vi "Create Oneof Protobuf To Field Name.vi"(8 "error in (no error)":errorcluster, 10 "message element metadata":T1={"Field Name"="nested_message_2", "Embedded Message Name"="echo_array_NestedMessage2", "Protobuf Index"=3, "MessageElementType"=enum."MessageValue", "Repeated"=FALSE, "Is in Oneof"=TRUE, "Oneof Container Name"="echo_array_NestedMessage_union"}, 11 "class in":refnum<vi>) -> (0 "error out":errorcluster, 3 "class out":refnum<vi>)   [LabVIEW 2019, in "gRPC Template Creation Utility.lvlib"]
uses:
  gRPC Template Creation Utility.lvlib
  TypeDefs/Message Element Metadata (Scripting).ctl
  TypeDefs/Message Element Type.ctl
  <vilib>/Utility/traverseref.llb/TRef TravTarget.ctl
  <vilib>/Utility/traverseref.llb/VI Scripting - Traverse.lvlib
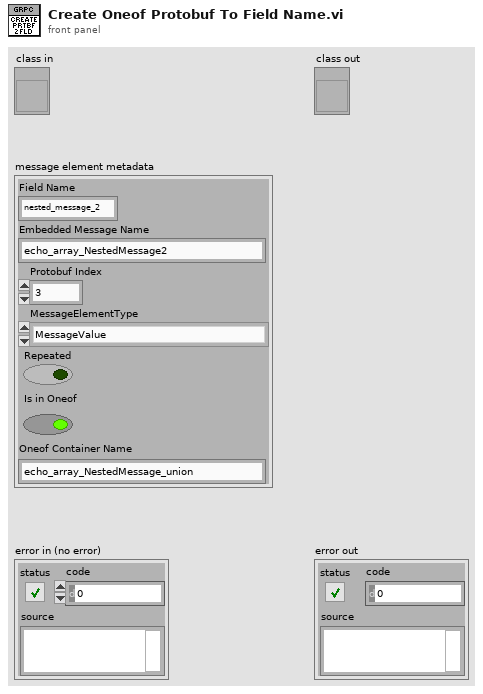
[diagram p1: front panel]
types:
  T1 = typedef "gRPC Template Creation Utility.lvlib/Message Element Metadata (Scripting).ctl" = cluster{"Field Name":string, "Embedded Message Name":string, "Protobuf Index":i32, "MessageElementType":T2, "Repeated":bool, "Is in Oneof":bool, "Oneof Container Name":string}
  T2 = typedef "gRPC Template Creation Utility.lvlib/Message Element Type.ctl" = enum32{"Int32Value", "FloatValue", "DoubleValue", "BoolValue", "StringValue", "MessageValue", "Int64Value", "UInt32Value", "UInt64Value", "EnumValue", "Bytes", "Fixed64", "Fixed32", "SFixed64", "SFixed32", "SInt64", "SInt32"}
  T3 = typedef "TRef TravTarget.ctl" = enum16{"FP", "BD", "Other"}
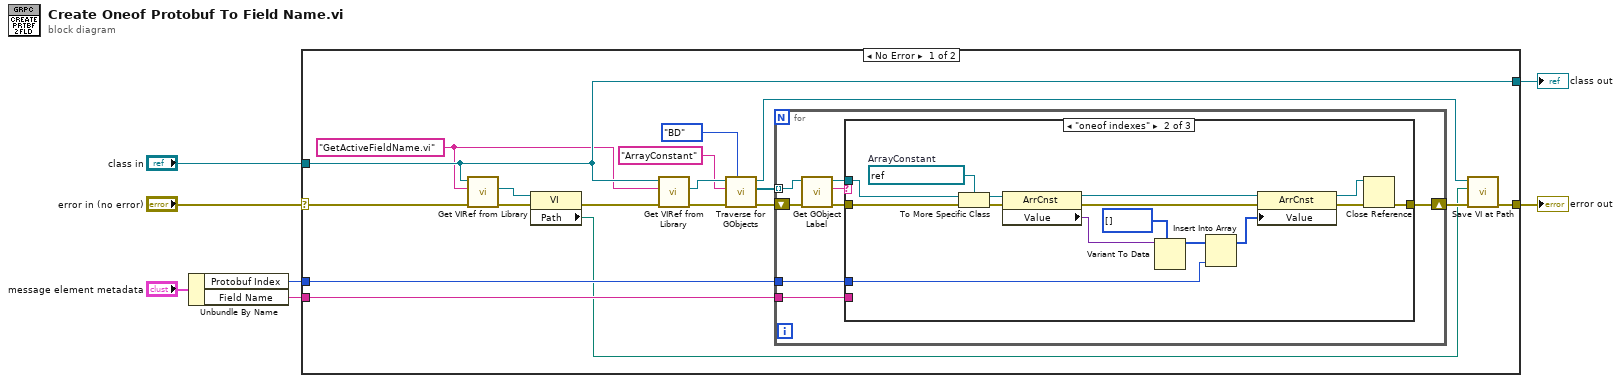
[diagram p0: block diagram]
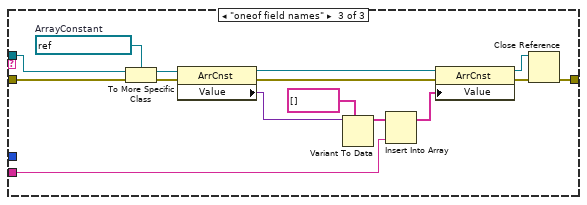
[diagram p3: hidden frame]
diagram:
  n1 = Unbundle By Name("message element metadata") -> ("Protobuf Index"=w1:i32, "Field Name"=w2:string)
  n2 = case shown="No Error" "error in (no error)" {
    selector: "error in (no error)" -> [w9 w65]
    tunnel: "class in" -> [w10 w66]
    tunnel: w1 -> [w21 _]
    tunnel: w2 -> [w20 _]
    tunnel: [w14 w65] -> w6
    tunnel: [w10 w66] -> w5
    frame No Error {
      w8 = "GetActiveFieldName.vi"
      n3 = call "Get VIRef from Library.vi"("error in (no error)"=w9, "item name"=w8, "library in"=w10) -> ("error out"=w12:errorcluster, "vi"=w11:refnum<vi>)  [unwired: 5 in, 2 out]
      n4 = property class="VI"(reference=w11, error in=w12) -> (error out=w25:errorcluster, "Path"=w13:path)  [unwired: 1 out]
      n5 = call "Get VIRef from Library.vi"("error in (no error)"=w25, "item name"=w8, "library in"=w10) -> ("error out"=w18:errorcluster, "vi"=w23:refnum<vi>)  [unwired: 5 in, 2 out]
      n6 = call <vilib>:"Traverse for GObjects.vi"("Traverse Target"=TRef_TravTarget."BD", "error in (no error)"=w18, "Class Name"="ArrayConstant", "VI Refnum"=w23) -> ("error out"=w19:errorcluster, "References"=w24:refnum<vi>[], "dup VI Refnum"=w16:refnum<vi>)  [unwired: 4 in, 1 out]
      n7 = for {
        tunnel: w24 -> [w33] mode=indexing
        tunnel: w21 -> [w30]
        tunnel: w20 -> [w29]
        shift-right: [w28] -> w15
        shift-left: w19 -> [w26]
        n8 = call <vilib>:"Get GObject Label.vi"("error in (no error)"=w26, "GObject"=w33) -> ("error out"=w27:errorcluster, "Object Label"=w32:string, "dup GObject"=w31:refnum<vi>)  [unwired: 5 in, 2 out]
        n9 = case shown="\"oneof indexes\"" w32 {
          tunnel: w31 -> [_ w49 w56]
          tunnel: w30 -> [_ w43 _]
          tunnel: w29 -> [_ _ w55]
          tunnel: [w34 w37 w52] -> w28
          tunnel: w27 -> [w34 w35 w51]
          frame Default {
          }
          frame "oneof indexes" {
            w48 = refnum<vi> refnum  # ArrayConstant
            n10 = To More Specific Class(target class=w48, reference=w49, error in=w35) -> (specific class reference=w47:refnum<vi>, error out=w41:errorcluster)
            n11 = property class="ArrCnst"(reference=w47, error in=w41) -> (reference out=w46:refnum<vi>, error out=w40:errorcluster, "Value"=w45:variant)
            n12 = Variant To Data(type=i32[] [], Variant=w45) -> (data=w36:i32[])  [unwired: 1 in, 1 out]
            n13 = Insert Into Array(array=w36, new element=w43) -> (w42:i32[])  [unwired: 1 in]
            n14 = property class="ArrCnst"(reference=w46, error in=w40, "Value"=w42) -> (reference out=w38:refnum<vi>, error out=w39:errorcluster)
            n15 = Close Reference(reference=w38, error in (no error)=w39) -> (error out=w37:errorcluster)
          }
          frame "oneof field names" {
            w64 = refnum<vi> refnum  # ArrayConstant
            n16 = To More Specific Class(target class=w64, reference=w56, error in=w51) -> (specific class reference=w63:refnum<vi>, error out=w58:errorcluster)
            n17 = property class="ArrCnst"(reference=w63, error in=w58) -> (reference out=w62:refnum<vi>, error out=w57:errorcluster, "Value"=w61:variant)
            n18 = Variant To Data(type=string[] [], Variant=w61) -> (data=w50:string[])  [unwired: 1 in, 1 out]
            n19 = Insert Into Array(array=w50, new element=w55) -> (w59:string[])  [unwired: 1 in]
            n20 = property class="ArrCnst"(reference=w62, error in=w57, "Value"=w59) -> (reference out=w54:refnum<vi>, error out=w53:errorcluster)
            n21 = Close Reference(reference=w54, error in (no error)=w53) -> (error out=w52:errorcluster)
          }
        }
      }
      n22 = call "Save VI at Path.vi"("error in (no error)"=w15, "Path"=w13, "VI in"=w16) -> ("error out"=w14:errorcluster)  [unwired: 6 in, 2 out]
    }
    frame Error {
    }
  }
  "error out" <- w6
  "class out" <- w5
